vi "VIH Project Tree - Item Type to Palette Item Type.vi"(11 "Tree Item Type":T2) -> (2 "PolyVI Instance VI":bool, 3 "Item/File Type":T1)   [LabVIEW 2014]
doc: "::: VI Helpeks :::\nCopyright (c) 2000-2026 Konstantin Shifershteyn. All rights reserved."
uses:
  VIH Project Tree Typedef - Tree Item Type.ctl
  _VIH HelpGen - Palette.llb/VIH HelpGen Typedef - Palette - Item Type Enum.ctl
panel:
  # "VI Helpeks\nCopyright (c) 2012-2026 Konstantin Shifershteyn"
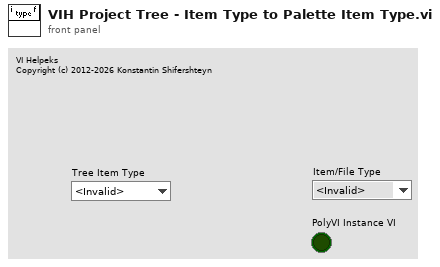
[diagram p1: front panel]
types:
  T1 = typedef "VIH HelpGen Typedef - Palette - Item Type Enum.ctl" = enum32{"<Invalid>", "<unknown>", "VI", "Menu", "LV Func", "Express VI", "Poly VI", "CTL", "HTML"}
  T2 = typedef "VIH Project Tree Typedef - Tree Item Type.ctl" = enum32{"<Invalid>", "Project", "Proj Files", "Proj Rules", "File Group", "Rule Group", "Any File", "LV Func", ".mnu", ".mnu (dyn)", ".vi", ".vi (dyn)", ".vit", ".vit (dyn)", ".ctl", ".ctl (dyn)", ".ctt", ".ctt (dyn)", "polyVI", "polyVI (dyn)", "expVI", "expVI (dyn)", "HTML", "PolyVI Inst"}
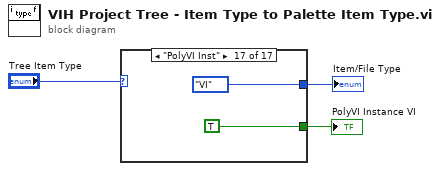
[diagram p0: block diagram]
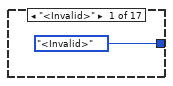
[diagram p2: hidden frame]
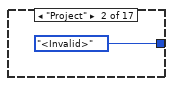
[diagram p3: hidden frame]
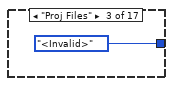
[diagram p4: hidden frame]
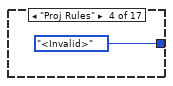
[diagram p5: hidden frame]
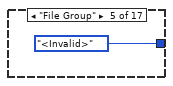
[diagram p6: hidden frame]
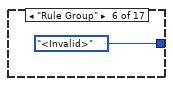
[diagram p7: hidden frame]
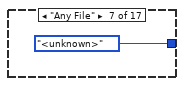
[diagram p8: hidden frame]
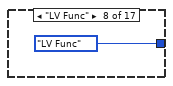
[diagram p9: hidden frame]
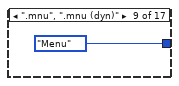
[diagram p10: hidden frame]
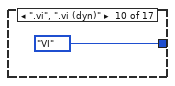
[diagram p11: hidden frame]
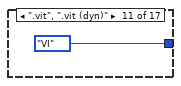
[diagram p12: hidden frame]
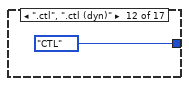
[diagram p13: hidden frame]
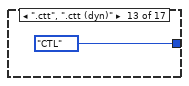
[diagram p14: hidden frame]
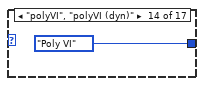
[diagram p15: hidden frame]
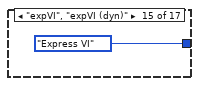
[diagram p16: hidden frame]
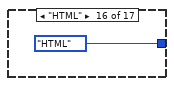
[diagram p17: hidden frame]
diagram:
  n1 = case shown="\"PolyVI Inst\"" "Tree Item Type" {
    tunnel: [VIH_HelpGen_Typedef_-_Palette_-_Item_Type_Enum."<Invalid>" ("File Type") VIH_HelpGen_Typedef_-_Palette_-_Item_Type_Enum."<Invalid>" ("File Type") VIH_HelpGen_Typedef_-_Palette_-_Item_Type_Enum."<Invalid>" ("File Type") VIH_HelpGen_Typedef_-_Palette_-_Item_Type_Enum."<Invalid>" ("File Type") VIH_HelpGen_Typedef_-_Palette_-_Item_Type_Enum."<Invalid>" ("File Type") VIH_HelpGen_Typedef_-_Palette_-_Item_Type_Enum."<Invalid>" ("File Type") VIH_HelpGen_Typedef_-_Palette_-_Item_Type_Enum."<unknown>" ("File Type") VIH_HelpGen_Typedef_-_Palette_-_Item_Type_Enum."LV Func" ("File Type") VIH_HelpGen_Typedef_-_Palette_-_Item_Type_Enum."Menu" ("File Type") VIH_HelpGen_Typedef_-_Palette_-_Item_Type_Enum."VI" ("File Type") VIH_HelpGen_Typedef_-_Palette_-_Item_Type_Enum."VI" ("File Type") VIH_HelpGen_Typedef_-_Palette_-_Item_Type_Enum."CTL" ("File Type") VIH_HelpGen_Typedef_-_Palette_-_Item_Type_Enum."CTL" ("File Type") VIH_HelpGen_Typedef_-_Palette_-_Item_Type_Enum."Poly VI" ("File Type") VIH_HelpGen_Typedef_-_Palette_-_Item_Type_Enum."Express VI" ("File Type") VIH_HelpGen_Typedef_-_Palette_-_Item_Type_Enum."HTML" ("File Type") VIH_HelpGen_Typedef_-_Palette_-_Item_Type_Enum."VI" ("File Type")] -> w2
    tunnel: [_ _ _ _ _ _ _ _ _ _ _ _ _ _ _ _ TRUE] -> w1
    frame "<Invalid>" {
    }
    frame "Project" {
    }
    frame "Proj Files" {
    }
    frame "Proj Rules" {
    }
    frame "File Group" {
    }
    frame "Rule Group" {
    }
    frame "Any File" {
    }
    frame "LV Func" {
    }
    frame ".mnu", ".mnu (dyn)" {
    }
    frame ".vi", ".vi (dyn)" {
    }
    frame ".vit", ".vit (dyn)" {
    }
    frame ".ctl", ".ctl (dyn)" {
    }
    frame ".ctt", ".ctt (dyn)" {
    }
    frame "polyVI", "polyVI (dyn)" {
    }
    frame "expVI", "expVI (dyn)" {
    }
    frame "HTML" {
    }
    frame "PolyVI Inst" {
    }
  }
  "Item/File Type" <- w2
  "PolyVI Instance VI" <- w1
